vi "Create.vi"(8 "error in (no error)":errorcluster, 11 "Identifier (ID, IP etc)":string) -> (0 "error out":errorcluster, 3 "Camera":refnum<class "Camera.lvclass">)   [LabVIEW 2020, in "Camera.lvclass"]
doc: "Create a camera instance based on an identifier such as the camera ID or IP address. This will attempt to connect to the camera and return an error if the camera is not available."
uses:
  Camera.lvclass
  Disconnected Registration.ctl
  Streaming Registation.ctl
  Stream User Events.ctl
  Camera.lvclass/Camera.ctl
  bin/gindustrialcam_32-1.dll
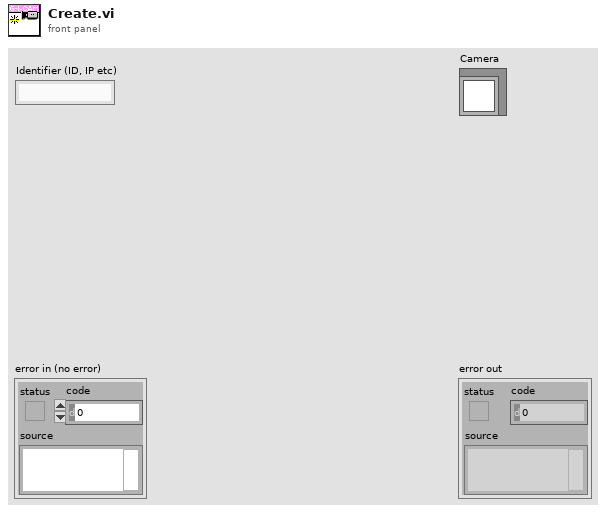
[diagram p1: front panel]
types:
  T1 = typedef "Camera.lvclass/Streaming Registation.ctl" = cluster{"Streaming Events":refnum<event-registration>, "User Events":T2}
  T2 = typedef "Camera.lvclass/Stream User Events.ctl" = cluster{"Stopped":refnum<user-event>, "Errors":refnum<user-event>}
  T3 = typedef "Camera.lvclass/Disconnected Registration.ctl" = cluster{"Disconnected":refnum<event-registration>, "User Event":refnum<user-event>}
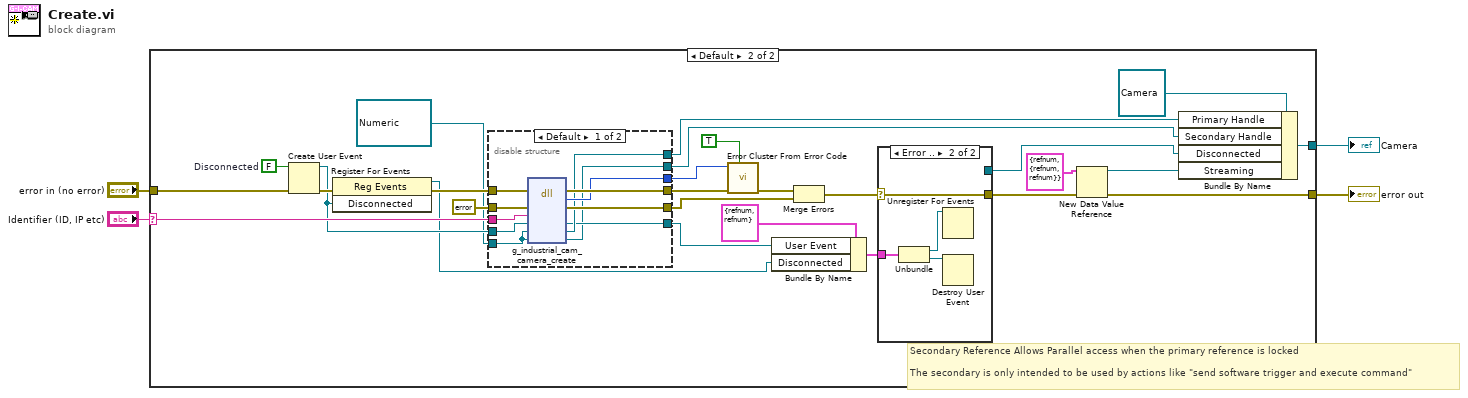
[diagram p0: block diagram]
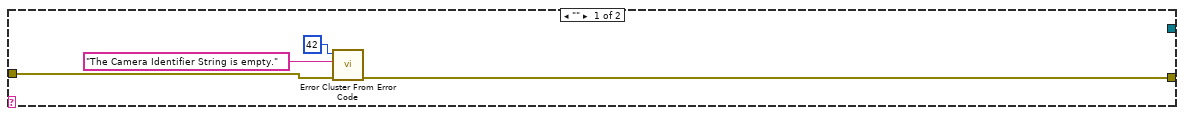
[diagram p2: hidden frame]
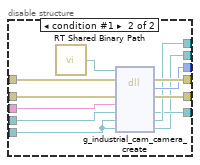
[diagram p3: hidden frame]
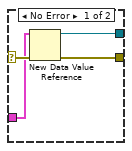
[diagram p4: hidden frame]
diagram:
  n1 = case shown="Default" "Identifier (ID, IP etc)" {
    selector: "Identifier (ID, IP etc)" -> [_ w29]
    tunnel: "error in (no error)" -> [w8 w24]
    tunnel: [w7 w12] -> w3
    tunnel: [_ w28] -> w1
    frame "" {
      n2 = call <vilib>:"Error Cluster From Error Code.vi"("error in (no error)"=w8, "error message (\"\")"="The Camera Identifier String is empty." ("error message (\"\")"), "error code (0)"=42) -> ("error out"=w7:errorcluster)  [unwired: 6 in]
    }
    frame Default {
      w26 = FALSE  # Disconnected
      # "Secondary Reference Allows Parallel access when the primary reference is locked\n\nThe secondary is only intended to be used by actions like \"send software trigger and execute command\""
      n3 = Create User Event(user event datatype=w26, error in=w24) -> (user event=w19:refnum<user-event>, error out=w23:errorcluster)
      n4 = register-events(error in=w23, w19) -> (reference out=w11:refnum<event-registration>, error out=w25:errorcluster)  [unwired: 1 in]
      n5 = disable-structure shown="Default" {
        disable-tunnel: [w46 w58] -> w35
        disable-tunnel: [w45 w57] -> w34
        disable-tunnel: [w44 w56] -> w32
        disable-tunnel: w29 -> [w43 w55]
        disable-tunnel: errorcluster {"status"=FALSE, "code"=0, "source"=""} ("error constant") -> [w42 w54]
        disable-tunnel: w25 -> [w41 w53]
        disable-tunnel: [w40 w52] -> w21
        disable-tunnel: w19 -> [w39 w51]
        disable-tunnel: [w38 w50] -> w17
        disable-tunnel: refnum<data-value> refnum ("data value reference") -> [w37 w49]
        disable-tunnel: [w36 w48] -> w9
        frame condition #0 (active) {
          n6 = dll-call lib="C:/serenial/lib/g-industrial-camera/LabVIEW/g_industrial_cam/bin/gindustrialcam_*-1.*" fn="g_industrial_cam_camera_create"(error in=w41, "err"=w42, "Identifier"=w43, "disconnected_user_event"=w39, "primary_edvr"=w37, "secondary_edvr"=w37) -> (error out=w46:errorcluster, "Mg_Error"=w45:i32, "err"=w44:errorcluster, "disconnected_user_event"=w38:refnum<user-event>, "primary_edvr"=w40:refnum<data-value>, "secondary_edvr"=w36:refnum<data-value>)  [unwired: 3 in, 1 out]
        }
        frame condition #1 {
          n7 = call "RT Shared Binary Path.vi"() -> ("Path"=w47:path)
          n8 = dll-call lib="C:/serenial/lib/g-industrial-camera/LabVIEW/g_industrial_cam/bin/gindustrialcam_*-1.*" fn="g_industrial_cam_camera_create"(path in=w47, error in=w53, "err"=w54, "Identifier"=w55, "disconnected_user_event"=w51, "primary_edvr"=w49, "secondary_edvr"=w49) -> (error out=w58:errorcluster, "Mg_Error"=w57:i32, "err"=w56:errorcluster, "disconnected_user_event"=w50:refnum<user-event>, "primary_edvr"=w52:refnum<data-value>, "secondary_edvr"=w48:refnum<data-value>)  [unwired: 2 in, 1 out]
        }
      }
      n9 = call <vilib>:"Error Cluster From Error Code.vi"("show call chain? (False)"=TRUE, "error in (no error)"=w35, "error code (0)"=w34) -> ("error out"=w33:errorcluster)  [unwired: 6 in]
      n10 = Bundle By Name(cluster=T3 {"Disconnected"=refnum, "User Event"=refnum} ("Disconnected Data"), "User Event"=w17, "Disconnected"=w11) -> (w18:T3)
      n11 = Merge Errors(w33, w32) -> (w22:errorcluster)
      n12 = case shown="Error .." w22 {
        selector: w22 -> [w62 w66]
        tunnel: w18 -> [w61 w65]
        tunnel: [w60 w66] -> w16
        tunnel: [w59 _] -> w13
        frame No Error {
          n13 = New Data Value Reference(data value=w61, error in=w62) -> (data value reference=w59:refnum<data-value>, error out=w60:errorcluster)
        }
        frame Error {
          n14 = Unbundle(w65) -> ("Disconnected"=w63:refnum<event-registration>, "User Event"=w64:refnum<user-event>)
          n15 = Unregister For Events(event registration refnum=w63) -> ()  [unwired: 1 in, 1 out]
          n16 = Destroy User Event(user event=w64) -> ()  [unwired: 1 in, 1 out]
        }
      }
      n17 = New Data Value Reference(data value=T1 {"Streaming Events"=refnum, "User Events"={"Stopped"=refnum, "Errors"=refnum}} ("Streaming Data"), error in=w16) -> (data value reference=w14:refnum<data-value>, error out=w12:errorcluster)
      n18 = Bundle By Name(cluster=refnum<class "Camera.lvclass"> refnum ("Camera out"), "Primary Handle"=w21, "Secondary Handle"=w9, "Disconnected"=w13, "Streaming"=w14) -> (w28:refnum<class "Camera.lvclass">)
    }
  }
  "error out" <- w3
  "Camera" <- w1
